vi "Take_Path.vi"(10 "组合框":T1="路径1") -> (2 "Your_Path":path)   [LabVIEW 2025, in "Path_management.lvclass"]
uses:
  Path_management.lvclass
  Register_path.ctl
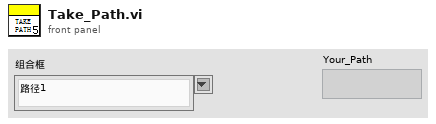
[diagram p1: front panel]
types:
  T1 = typedef "Path_management.lvclass/Register_path.ctl" = string
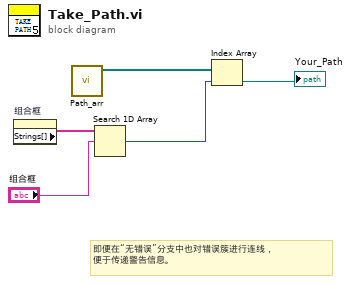
[diagram p0: block diagram]
diagram:
  # "即便在“无错误”分支中也对错误簇进行连线，\n便于传递警告信息。"
  n1 = property on="组合框" class="CmbBox (严格)"() -> ("Strings[]"=w5:string[])  [unwired: 2 in, 2 out]
  n2 = call "Path_arr.vi"() -> ("Path-arr 2"=w2:path[])  [unwired: 11 in]
  n3 = Search 1D Array(1D array=w5, element="组合框") -> (index of element=w3:i32)  [unwired: 1 in]
  n4 = Index Array(array=w2, index=w3) -> (element=→"Your_Path":path)
